vi "Flush Table.vi"(8 "error in":errorcluster, 11 "UI GUID":string) -> (0 "error out":errorcluster)   [LabVIEW 2025, in "CAN-LIN Raw Bus Capture UI.lvlib"]
uses:
  CAN-LIN Raw Bus Capture UI.lvlib
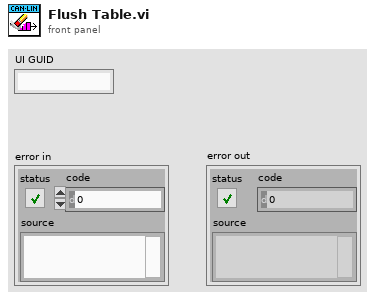
[diagram p1: front panel]
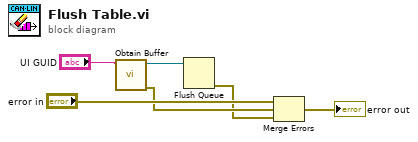
[diagram p0: block diagram]
diagram:
  n1 = call "Obtain Buffer.vi"("UI GUID"="UI GUID") -> ("error out"=w3:errorcluster, "Table Queue"=w4:refnum<queue>)  [unwired: 9 in]
  n2 = Flush Queue(queue=w4) -> (error out=w2:errorcluster)  [unwired: 1 in, 2 out]
  n3 = Merge Errors("error in", w3, w2) -> (→"error out":errorcluster)
